vi "时频联合分析.vi"() -> ()   [LabVIEW 2021]
doc: "本VI是为《我和LabVIEW》一书编写的示例。\n关于本书的介绍请参考网页：\nhttp://ruanqizhen.spaces.live.com/blog/cns!5852D4F797C53FB6!4310.entry"
uses:
  <vilib>/measure/maspectr.llb/FFT Power Spectrum and PSD for 1 Chan.vi
  <vilib>/measure/NI_MAPro.lvlib
panel:
  out "Waveform Graph":cluster{"f0":dbl, "df":dbl, "magnitude":dbl[]}(graph)
  out "Intensity Graph":dbl[][](graph)
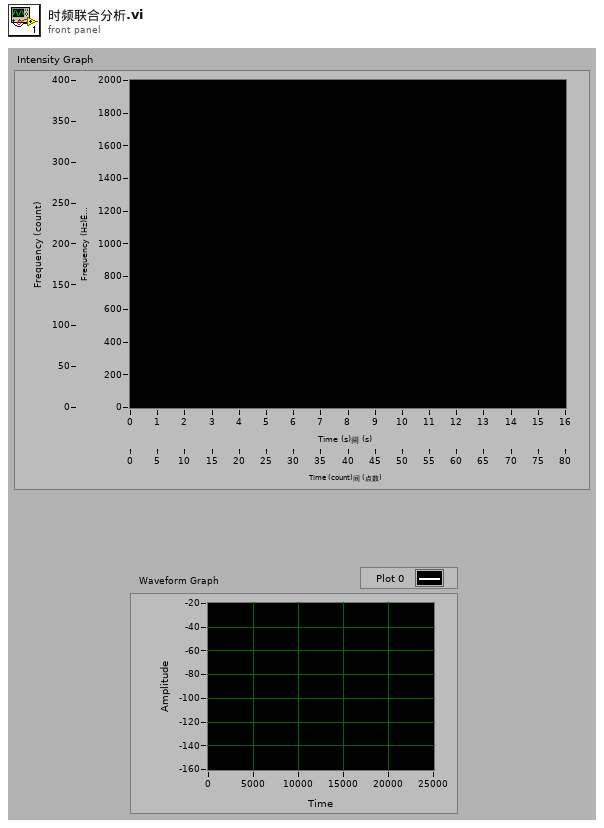
[diagram p1: front panel]
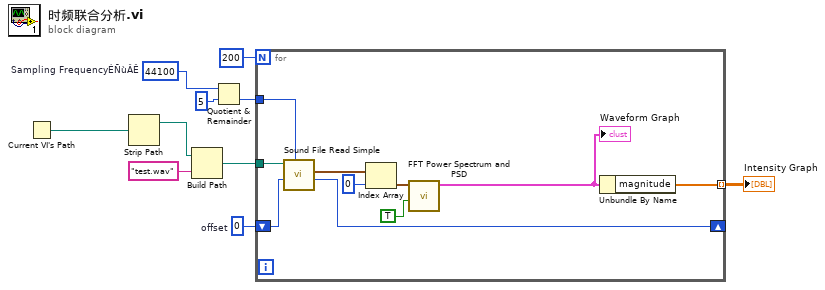
[diagram p0: block diagram]
diagram:
  w4 = 0  # offset
  w2 = 44100  # Sampling FrequencyÉÑùÂÊ
  n1 = Current VI's Path() -> (path=w9:path)
  n2 = Strip Path(path=w9) -> (stripped path=w10:path)  [unwired: 1 out]
  n3 = Build Path(base path=w10, name or relative path="test.wav" ("名称或相对路径")) -> (appended path=w5:path)
  n4 = Quotient & Remainder(x=w2, y=5) -> (floor(x/y)=w1:i32)  [unwired: 1 out]
  n5 = for {
    N: 200 -> [_]
    tunnel: w5 -> [w20]
    tunnel: [w19] -> w6 mode=indexing
    shift-right: [w15] -> _
    shift-left: w4 -> [w16]
    tunnel: w1 -> [w14]
    n6 = call <vilib>:"Sound File Read Simple.vi"("number of samples/ch (-1: all)"=w14, "position offset"=w16, "path"=w20) -> ("offset"=w15:i32, "data"=w18:waveform(dbl)[])  [unwired: 2 in, 5 out]
    n7 = Index Array(array=w18, index=0) -> (element=w13:waveform(dbl))
    n8 = call-poly <vilib>:"FFT Power Spectrum and PSD.vi"("dB On (F)"=TRUE, "time signal"=w13) -> ("Power Spectrum / PSD"=w11:cluster{"f0":dbl, "df":dbl, "magnitude":dbl[]})  [unwired: 6 in, 3 out]
    "Waveform Graph" <- w11
    n9 = Unbundle By Name "Unbundle By Name"(w11) -> ("magnitude"=w19:dbl[])
  }
  "Intensity Graph" <- w6
